vi "Read Blackboard Reference.vi"(8 "error in (no error)":errorcluster, 11 "CIF_Iceoryx_BB in":refnum<class "CIF_Iceoryx_BB.lvclass">) -> (0 "error out":errorcluster, 2 "BB Refnum":T1 {"refnum" format="%.0x"}, 3 "CIF_Iceoryx_BB out":refnum<class "CIF_Iceoryx_BB.lvclass">)   [LabVIEW 2021, in "CIF_Iceoryx_BB.lvclass"]
uses:
  CIF_Iceoryx_BB.lvclass
  CIF_Iceoryx_BB.lvclass/CIF_Iceoryx_BB.ctl
  <vilib>/CIF Foundation/CIF Iceoryx/Refnum/Typedef/BB Refnum.ctl
  <vilib>/CIF Foundation/CIF Iceoryx/Iceoryx.lvlib
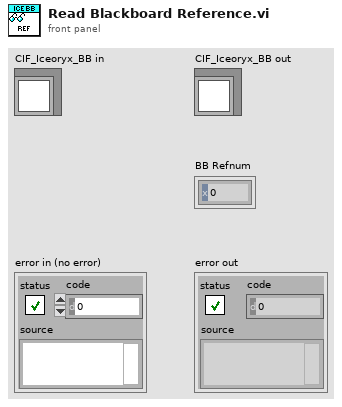
[diagram p1: front panel]
types:
  T1 = typedef "Iceoryx.lvlib/BB Refnum.ctl" = cluster{"refnum":u64, "BB":enum8{"bb"}}
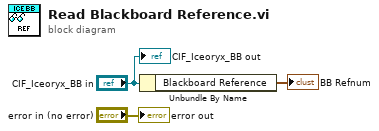
[diagram p0: block diagram]
diagram:
  n1 = Unbundle By Name("CIF_Iceoryx_BB in") -> ("Blackboard Reference"=→"BB Refnum":T1)
  "error out" <- "error in (no error)"
  "CIF_Iceoryx_BB out" <- "CIF_Iceoryx_BB in"
